vi "VHist - Multiple DBL history to spreadsheet string.vi"(4 "data format (%.3f)":string="%.3f", 5 "history headers":string[](array[string]), 6 "time stamp format (%c)":string="%c", 7 "time stamp header":string="Time stamp", 8 "error in":errorcluster, 9 "empty for NaN (F)":bool, 10 "multiple history data":cluster{"history data":dbl[]}[](array[cluster]), 11 "time stamps":dbl[](array[numeric]) format="%<%H:%M:%S%2u\n%d/%m/%Y>T") -> (0 "error out":errorcluster, 3 "spreadsheet string":string)   [LabVIEW 2021]
doc: "The VI converts multiple DBL history to spreadsheet string.\n\nIt is possible to specify format of numbers and time stamps. Optionally, the VI can replace NaN with an empty string. In addition, column headers can be added to the output string.\n\n::: CalcExpress Toolkit :::\nCopyright (c) 2000-2026 Konstantin Shifershteyn. All rights reserved."
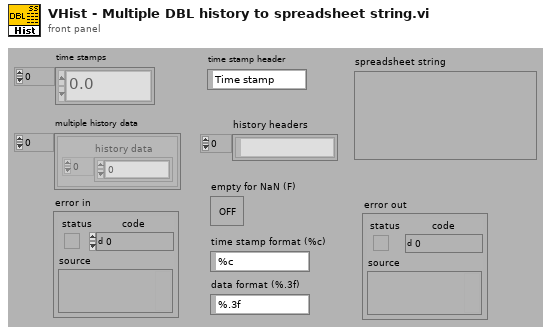
[diagram p1: front panel]
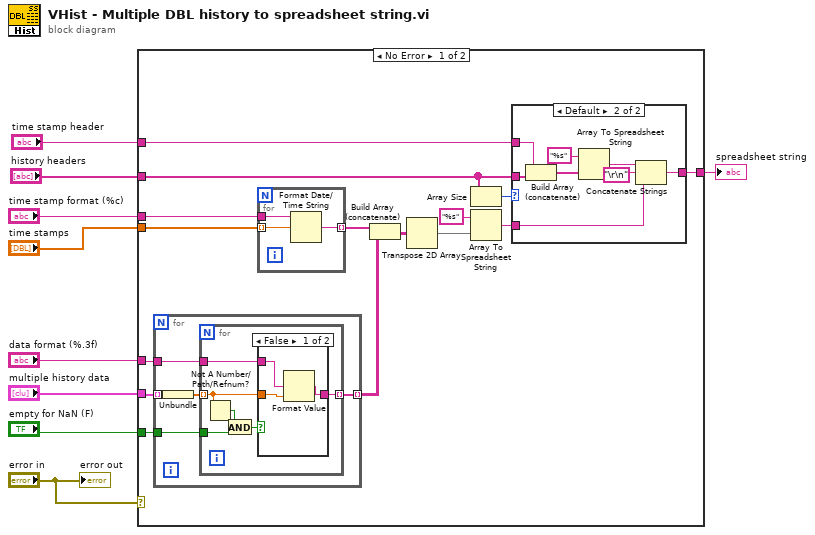
[diagram p0: block diagram]
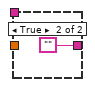
[diagram p2: hidden frame]
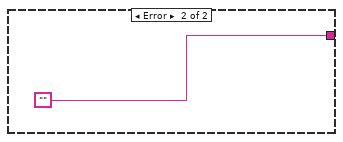
[diagram p4: hidden frame]
diagram:
  n1 = case shown="No Error" "error in" {
    tunnel: "time stamp format (%c)" -> [w21 _]
    tunnel: "time stamps" -> [w19 _]
    tunnel: "multiple history data" -> [w14 _]
    tunnel: [w18 ""] -> w5
    tunnel: "data format (%.3f)" -> [w13 _]
    tunnel: "empty for NaN (F)" -> [w15 _]
    tunnel: "time stamp header" -> [w11 _]
    tunnel: "history headers" -> [w10 _]
    frame No Error {
      n2 = for {
        tunnel: w14 -> [w29] mode=indexing
        tunnel: [w28] -> w12 mode=indexing
        tunnel: w13 -> [w26]
        tunnel: w15 -> [w25]
        n3 = Unbundle(w29) -> ("history data"=w27:dbl[])
        n4 = for {
          tunnel: [w35] -> w28 mode=indexing
          tunnel: w27 -> [w33] mode=indexing
          tunnel: w26 -> [w34]
          tunnel: w25 -> [w32]
          n5 = Not A Number/Path/Refnum?(number/path/refnum=w33) -> (NaN/Path/Refnum?=w31:bool)
          n6 = And(x=w31, y=w32) -> (x .and. y?=w30:bool)
          n7 = case shown="False" w30 {
            tunnel: [w38 ""] -> w35
            tunnel: w33 -> [w37 _]
            tunnel: w34 -> [w36 _]
            frame False {
              n8 = Format Value(format string=w36, value (0)=w37) -> (output string=w38:string)  [unwired: 1 in]
            }
            frame True {
            }
          }
        }
      }
      n9 = for {
        tunnel: w19 -> [w51] mode=indexing
        tunnel: w21 -> [w50]
        tunnel: [w49] -> w20 mode=indexing
        n10 = Format Date/Time String(time format string (%c)=w50, seconds (now)=w51) -> (date/time string=w49:string)  [unwired: 1 in]
      }
      n11 = Build Array (concatenate)(w20, w12) -> (w22:string[][])
      n12 = Transpose 2D Array(2D array=w22) -> (transposed array=w23:string[][])
      n13 = Array Size(array=w10) -> (size(s)=w16:i32)
      n14 = Array To Spreadsheet String(array=w23, 3:"%s" ("format string")) -> (spreadsheet string=w17:string)  [unwired: 1 in]
      n15 = case shown="Default" w16 {
        tunnel: w10 -> [_ w45]
        tunnel: [w40 w48] -> w18
        tunnel: w17 -> [w40 w47]
        tunnel: w11 -> [_ w46]
        frame 0 {
        }
        frame Default {
          n16 = Build Array (concatenate)(w46, w45) -> (w44:string[])
          n17 = Array To Spreadsheet String(array=w44, 3:"%s" ("format string")) -> (spreadsheet string=w42:string)  [unwired: 1 in]
          n18 = Concatenate Strings(w42, "\r\n", w47) -> (w48:string)
        }
      }
    }
    frame Error {
    }
  }
  "spreadsheet string" <- w5
  "error out" <- "error in"
